vi "FuncVI-PPulse.vi"(5 "InstanceRef":T2, 9 "arg list":T1[](array[typedef]) {"num" format="%.2f"}) -> (0 "error out":bool, 3 "result":T1 {"num" format="%.2f"})   [LabVIEW 2021]
doc: "::: CalcExpress Toolkit :::\nCopyright (c) 2000-2026 Konstantin Shifershteyn. All rights reserved."
uses:
  cetypes.llb/CalcExpress Function Argument Info.ctl
  cetypes.llb/CalcExpress Instance RefNum.ctl
  <vilib>/Analysis/NI_AALBase.lvlib
panel:
  in  "max arg num":i32=4
  in  "min arg num":i32
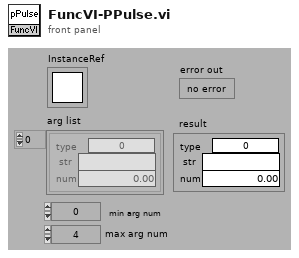
[diagram p1: front panel]
types:
  T1 = typedef "CalcExpress Function Argument Info.ctl" = cluster{"type":u32, "str":string, "num":dbl}
  T2 = typedef "CalcExpress Instance RefNum.ctl" = refnum<k1>
  T3 = enum8{"String", "DBL Number", "identifier", "1D Array of DBL", "2D Array of DBL", "CDB Number", "1D Array of CDB", "2D Array of CDB", "1D Array of String", "2D Array of String", "Unknown data type"}
  T4 = cluster{"index":i32, "type":enum8{"String", "DBL Number", "identifier", "1D Array of DBL", "2D Array of DBL", "CDB Number", "1D Array of CDB", "2D Array of CDB", "Unknown data type"}, "default num":dbl, "default str":string}[]
  T5 = cluster{"num list[0]":dbl, "num list[1]":dbl, "num list[2]":dbl, "num list[3]":dbl}
  T6 = cluster{"type":enum8{"String", "DBL Number", "identifier", "1D Array of DBL", "2D Array of DBL", "CDB Number", "1D Array of CDB", "2D Array of CDB", "1D Array of String", "2D Array of String", "Unknown data type"}, "data string":string, dbl}
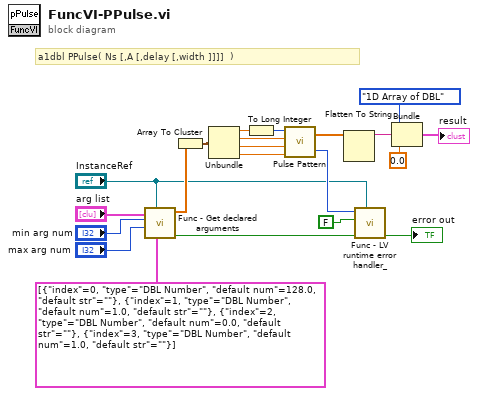
[diagram p0: block diagram]
diagram:
  # "a1dbl PPulse( Ns [,A [,delay [,width ]]]]  )"
  n1 = call "Func - Get declared arguments.vi"("arg descriptors"=T4 [{"index"=0, "type"=enum."DBL Number", "default num"=128.0, "default str"=""}, {"index"=1, "type"=enum."DBL Number", "default num"=1.0, "default str"=""}, {"index"=2, "type"=enum."DBL Number", "default num"=0.0, "default str"=""}, {"index"=3, "type"=enum."DBL Number", "default num"=1.0, "default str"=""}] ("args descriptors"), "InstanceRef"="InstanceRef", "max arg num"="max arg num", "min arg num"="min arg num", "arg list"="arg list") -> ("error out"=w11:bool, "num list"=w20:dbl[])  [unwired: 3 in, 2 out]
  n2 = Array To Cluster(array=w20) -> (cluster=w19:T5)
  n3 = Unbundle(w19) -> ("num list[0]"=w14:dbl, "num list[1]"=w8:dbl, "num list[2]"=w7:dbl, "num list[3]"=w6:dbl)
  n4 = To Long Integer(number=w14) -> (32bit integer=w13:i32)
  n5 = call <vilib>:"Pulse Pattern.vi"("width"=w6, "delay"=w7, "amplitude"=w8, "samples"=w13) -> ("error"=w12:i32, "Pulse Pattern"=w10:dbl[])
  n6 = Flatten To String(anything=w10) -> (data string=w9:string)  [unwired: 3 in, 2 out]
  n7 = call "Func - LV runtime error handler_.vi"("InstanceRef"="InstanceRef", "error in"=w11, "Gen CE error?"=FALSE, "LabVIEW error code"=w12) -> ("error out"=→"error out":bool)  [unwired: 7 in]
  n8 = Bundle("type"=T3."1D Array of DBL", "data string"=w9, 0.0) -> (→"result":T6)  [unwired: 1 in]
